vi "sftp_append.vi"() -> ()   [LabVIEW 2017]
doc: "Illustrates how to append to a file using SFTP."
uses:
  libssh2/libssh2_session_handshake_tcp.vi
  libssh2/libssh2_init_default.vi
  libssh2/libssh2_session_init_ex.vi
  <vilib>/Utility/tcp.llb/TCP Get Raw Net Object.vi
  libssh2/libssh2_session_handshake_socket.vi
  libssh2/libssh2_userauth_password_ex.vi
  libssh2/libssh2_sftp_open_ex.vi
  libssh2/libssh2_sftp_fstat_ex.vi
  libssh2/libssh2.lvlib
panel:
  out "file position before write":u64
  out "file position after write":u64
  out "filesize":u64
  out "file content":string
  in  "file":string="/"
  in  "append text":string="Lorem ipsum dolor sit amet, consetetur sadipscing elitr, sed diam nonumy eirmod tempor invidunt ut labore et dolore magna aliquyam erat, sed diam voluptua. At vero eos et accusam et justo duo dolores et ea rebum. Stet clita kasd gubergren, no sea takimata sanctus est Lorem ipsum dolor sit amet. Lorem ipsum dolor sit amet, consetetur sadipscing elitr, sed diam nonumy eirmod tempor invidunt ut labore et dolore magna aliquyam erat, sed diam voluptua. At vero eos et accusam et justo duo dolores et ea rebum. Stet clita kasd gubergren, no sea takimata sanctus est Lorem ipsum dolor sit amet. "
  out "error out":errorcluster
  in  "password":string
  in  "username":string
  in  "hostname":string
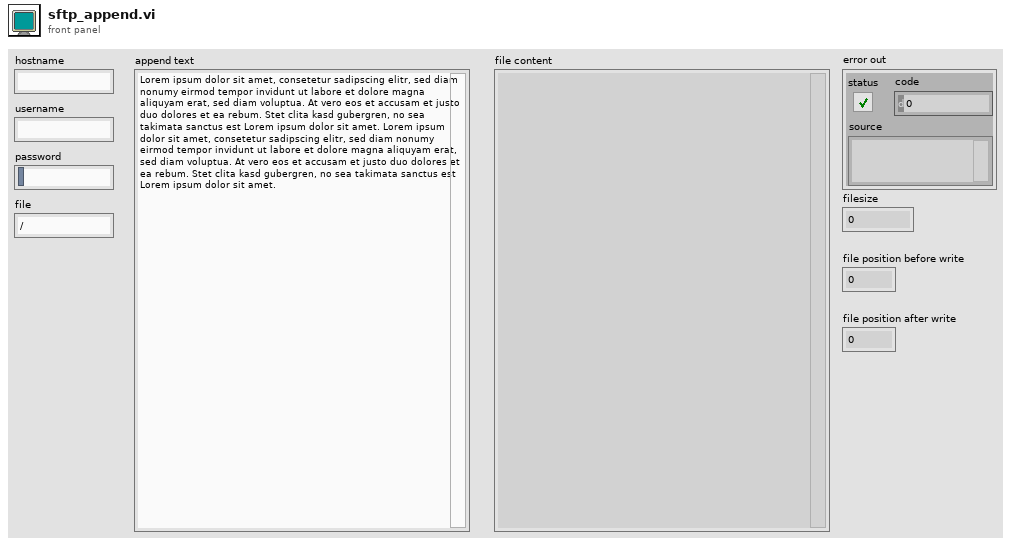
[diagram p1: front panel]
types:
  T1 = typedef "libssh2.lvlib/Session Refnum.ctl" = refnum<k1>
  T2 = typedef "libssh2.lvlib/SFTP Refnum.ctl" = refnum<k1>
  T3 = typedef "libssh2.lvlib/SFTP Handle Refnum.ctl" = refnum<k1>
  T4 = typedef "libssh2.lvlib/libssh2_sftp_attributes.ctl" = cluster{"flags":u32, "filesize":u64, "uid":u32, "gid":u32, "permissions":u32, "atime":u32, "mtime":u32}
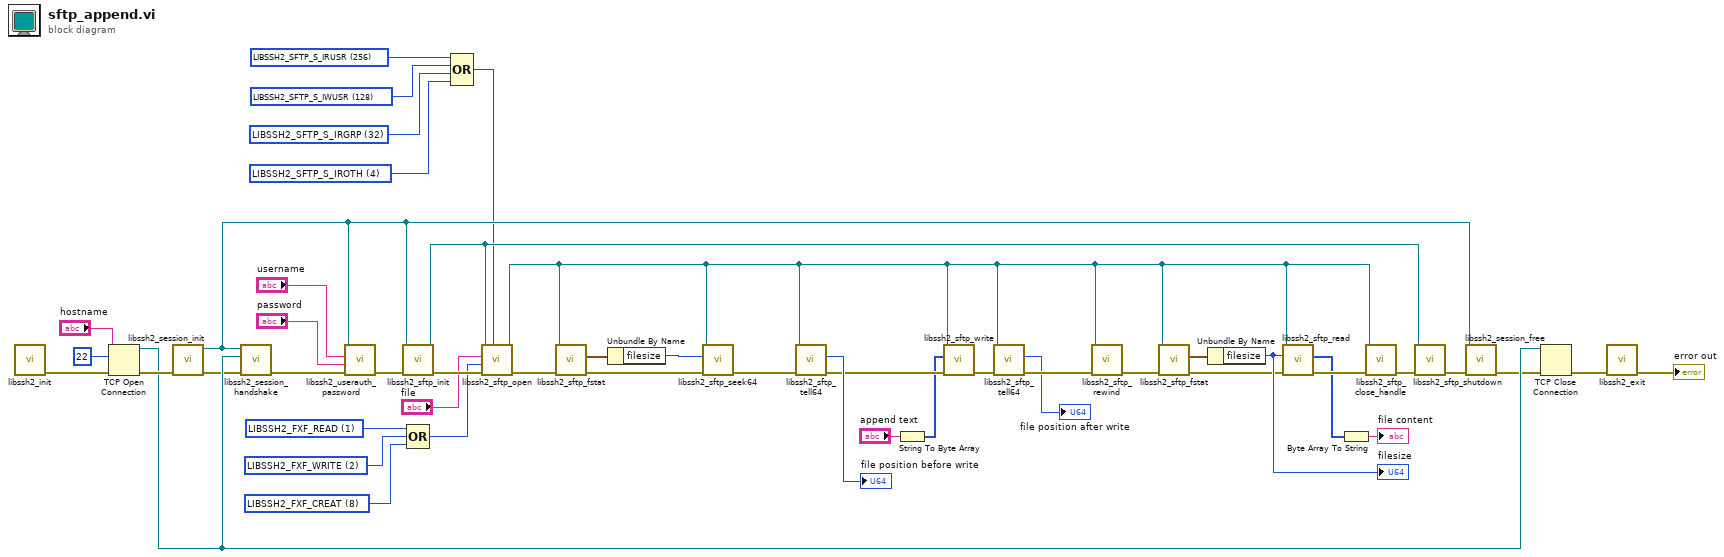
[diagram p0: block diagram]
diagram:
  w15 = u32 8 items=["LIBSSH2_FXF_READ"=1, "LIBSSH2_FXF_WRITE"=2, "LIBSSH2_FXF_APPEND"=4, "LIBSSH2_FXF_CREAT"=8, "LIBSSH2_FXF_TRUNC"=16, "LIBSSH2_FXF_EXCL"=32] ("flags")
  w23 = 4 items=["LIBSSH2_SFTP_S_IRWXU"=448, "LIBSSH2_SFTP_S_IRUSR"=256, "LIBSSH2_SFTP_S_IWUSR"=128, "LIBSSH2_SFTP_S_IXUSR"=64, "LIBSSH2_SFTP_S_IRWXG"=56, "LIBSSH2_SFTP_S_IRGRP"=32, "LIBSSH2_SFTP_S_IWGRP"=16, "LIBSSH2_SFTP_S_IXGRP"=8, "LIBSSH2_SFTP_S_IRWXO"=7, "LIBSSH2_SFTP_S_IROTH"=4, "LIBSSH2_SFTP_S_IWOTH"=2, "LIBSSH2_SFTP_S_IXOTH"=1] ("mode")
  w24 = 32 items=["LIBSSH2_SFTP_S_IRWXU"=448, "LIBSSH2_SFTP_S_IRUSR"=256, "LIBSSH2_SFTP_S_IWUSR"=128, "LIBSSH2_SFTP_S_IXUSR"=64, "LIBSSH2_SFTP_S_IRWXG"=56, "LIBSSH2_SFTP_S_IRGRP"=32, "LIBSSH2_SFTP_S_IWGRP"=16, "LIBSSH2_SFTP_S_IXGRP"=8, "LIBSSH2_SFTP_S_IRWXO"=7, "LIBSSH2_SFTP_S_IROTH"=4, "LIBSSH2_SFTP_S_IWOTH"=2, "LIBSSH2_SFTP_S_IXOTH"=1] ("mode")
  w25 = 128 items=["LIBSSH2_SFTP_S_IRWXU"=448, "LIBSSH2_SFTP_S_IRUSR"=256, "LIBSSH2_SFTP_S_IWUSR"=128, "LIBSSH2_SFTP_S_IXUSR"=64, "LIBSSH2_SFTP_S_IRWXG"=56, "LIBSSH2_SFTP_S_IRGRP"=32, "LIBSSH2_SFTP_S_IWGRP"=16, "LIBSSH2_SFTP_S_IXGRP"=8, "LIBSSH2_SFTP_S_IRWXO"=7, "LIBSSH2_SFTP_S_IROTH"=4, "LIBSSH2_SFTP_S_IWOTH"=2, "LIBSSH2_SFTP_S_IXOTH"=1] ("mode")
  w26 = 256 items=["LIBSSH2_SFTP_S_IRWXU"=448, "LIBSSH2_SFTP_S_IRUSR"=256, "LIBSSH2_SFTP_S_IWUSR"=128, "LIBSSH2_SFTP_S_IXUSR"=64, "LIBSSH2_SFTP_S_IRWXG"=56, "LIBSSH2_SFTP_S_IRGRP"=32, "LIBSSH2_SFTP_S_IWGRP"=16, "LIBSSH2_SFTP_S_IXGRP"=8, "LIBSSH2_SFTP_S_IRWXO"=7, "LIBSSH2_SFTP_S_IROTH"=4, "LIBSSH2_SFTP_S_IWOTH"=2, "LIBSSH2_SFTP_S_IXOTH"=1] ("mode")
  w28 = u32 2 items=["LIBSSH2_FXF_READ"=1, "LIBSSH2_FXF_WRITE"=2, "LIBSSH2_FXF_APPEND"=4, "LIBSSH2_FXF_CREAT"=8, "LIBSSH2_FXF_TRUNC"=16, "LIBSSH2_FXF_EXCL"=32] ("flags")
  w29 = u32 1 items=["LIBSSH2_FXF_READ"=1, "LIBSSH2_FXF_WRITE"=2, "LIBSSH2_FXF_APPEND"=4, "LIBSSH2_FXF_CREAT"=8, "LIBSSH2_FXF_TRUNC"=16, "LIBSSH2_FXF_EXCL"=32] ("flags")
  n1 = call-poly "libssh2_init.vi"() -> ("error out"=w47:errorcluster)  [unwired: 11 in]
  n2 = TCP Open Connection(address="hostname", remote port or service name=u16 22, error in (no error)=w47) -> (connection ID=w45:refnum<k5>, error out=w46:errorcluster)  [unwired: 2 in]
  n3 = call "libssh2_session_init.vi"("error in (no error)"=w46) -> ("error out"=w44:errorcluster, "session"=w37:T1)  [unwired: 9 in]
  n4 = call-poly "libssh2_session_handshake.vi"("error in (no error)"=w44, "tcp connection"=w45, "session"=w37) -> ("error out"=w48:errorcluster)  [unwired: 8 in]
  n5 = call "libssh2_userauth_password.vi"("error in (no error)"=w48, "password"="password", "username"="username", "session"=w37) -> ("error out"=w41:errorcluster)  [unwired: 7 in]
  n6 = call "libssh2_sftp_init.vi"("error in (no error)"=w41, "session"=w37) -> ("error out"=w33:errorcluster, "sftp"=w32:T2)  [unwired: 8 in]
  n7 = Compound Arithmetic op=OR(w29, w28, w15) -> (w27:u32)
  n8 = Compound Arithmetic op=OR(w26, w25, w24, w23) -> (w22:i32)
  n9 = call "libssh2_sftp_open.vi"("mode"=w22, "error in (no error)"=w33, "flags"=w27, "path"="file", "sftp"=w32) -> ("error out"=w21:errorcluster, "sftp handle"=w3:T3)  [unwired: 5 in]
  n10 = call "libssh2_sftp_fstat.vi"("error in (no error)"=w21, "sftp handle"=w3) -> ("error out"=w20:errorcluster, "attributes out"=w19:T4)  [unwired: 8 in]
  n11 = Unbundle By Name(w19) -> ("filesize"=w18:u64)
  n12 = call "libssh2_sftp_seek64.vi"("error in (no error)"=w20, "offset"=w18, "sftp handle"=w3) -> ("error out"=w5:errorcluster)  [unwired: 8 in]
  n13 = call "libssh2_sftp_tell64.vi"("error in (no error)"=w5, "sftp handle"=w3) -> ("error out"=w4:errorcluster, "offset"=→"file position before write":u64)  [unwired: 8 in]
  n14 = String To Byte Array(string="append text") -> (unsigned byte array=w2:u8[])
  n15 = call "libssh2_sftp_write.vi"("error in (no error)"=w4, "buffer"=w2, "sftp handle"=w3) -> ("error out"=w17:errorcluster)  [unwired: 7 in, 1 out]
  n16 = call "libssh2_sftp_tell64.vi"("error in (no error)"=w17, "sftp handle"=w3) -> ("error out"=w8:errorcluster, "offset"=→"file position after write":u64)  [unwired: 8 in]
  n17 = call "libssh2_sftp_rewind.vi"("error in (no error)"=w8, "sftp handle"=w3) -> ("error out"=w11:errorcluster)  [unwired: 9 in]
  n18 = call "libssh2_sftp_fstat.vi"("error in (no error)"=w11, "sftp handle"=w3) -> ("error out"=w10:errorcluster, "attributes out"=w13:T4)  [unwired: 8 in]
  n19 = Unbundle By Name(w13) -> ("filesize"=w12:u64)
  "filesize" <- w12
  n20 = call "libssh2_sftp_read.vi"("error in (no error)"=w10, "buffer maxlen"=w12, "sftp handle"=w3) -> ("error out"=w14:errorcluster, "buffer"=w9:u8[])  [unwired: 6 in, 1 out]
  n21 = Byte Array To String(unsigned byte array=w9) -> (string=→"file content":string)
  n22 = call "libssh2_sftp_close_handle.vi"("error in (no error)"=w14, "sftp handle"=w3) -> ("error out"=w30:errorcluster)  [unwired: 9 in]
  n23 = call "libssh2_sftp_shutdown.vi"("error in (no error)"=w30, "sftp"=w32) -> ("error out"=w34:errorcluster)  [unwired: 9 in]
  n24 = call "libssh2_session_free.vi"("error in (no error)"=w34, "session"=w37) -> ("error out"=w36:errorcluster)  [unwired: 9 in]
  n25 = TCP Close Connection(connection ID=w45, error in (no error)=w36) -> (error out=w35:errorcluster)  [unwired: 1 in, 1 out]
  n26 = call "libssh2_exit.vi"("error in (no error)"=w35) -> ("error out"=→"error out":errorcluster)  [unwired: 10 in]
